vi "Test Variant to Objects.vi"() -> ()   [LabVIEW 2021]
uses:
  Source/Support/Nodes/Leaves/Synch/With Values/WaitOn/bt_WaitOn_Synch_WithValues.lvclass
  <vilib>/ErrorRing/Error Ring.xnode
  <vilib>/Utility/error.llb/Error Cluster From Error Code.vi
  <vilib>/measure/NI_MABase.lvlib
  <vilib>/TSA/Abstract Data Classes/Abs_Types/Waveform/Abs_Waveform.lvclass
  <vilib>/TSA/Abstract Data Classes/Abs_Types/Boolean/Abs_Boolean.lvclass
  <vilib>/TSA/Abstract Data Classes/Abs_Types/I32 Integer/Abs_I32 Integer.lvclass
  <vilib>/TSA/Abstract Data Classes/Abs_Types/String/Abs_String.lvclass
  <vilib>/TSA/Omni-Bus/Local Bus/Local Bus.lvclass
  <vilib>/Utility/Data Type/Type Definitions/Data Type.ctl
  <vilib>/Utility/Data Type/NI_Data Type.lvlib
  <vilib>/TSA/Omni-Bus/Local Bus/Support/Tag List Type.ctl
  <vilib>/TSA/Omni-Bus/Omni-Bus/Omni_Bus.lvclass
  <vilib>/TSA/Abstract Data Classes/Abs_Types/Double Float/Abs_Double Float.lvclass
  <vilib>/TSA/Omni-Bus/Omni-Bus/Support/Get/Get DBL.vi
  <vilib>/TSA/Abstract Data Classes/Abs_Types/Time/Abs_Time.lvclass
  <vilib>/TSA/Abstract Data Classes/Abs_Types/Boolean/Simple Read.vi
  <vilib>/TSA/Abstract Data Classes/Abs_Types/I32 Integer/Simple Read.vi
  <vilib>/TSA/Abstract Data Classes/Abs_Types/String/Simple Read.vi
  <vilib>/TSA/Abstract Data Classes/Abs_Types/Waveform/Simple Read.vi
  <vilib>/TSA/Abstract Data Classes/Abs_Types/Time/Simple Read.vi
  <vilib>/TSA/Omni-Bus/Omni-Bus/Support/Write/Write DBL.vi
  <vilib>/TSA/Abstract Data Classes/Abs_Types/Double Float/Simple Read.vi
  C:/Program Files (x86)/National Instruments/LabVIEW 2021/vi.lib/TSA/Omni-Bus/Omni-Bus/Bus Access/Bus_Access.lvclass
  C:/Program Files (x86)/National Instruments/LabVIEW 2021/vi.lib/TSA/Abstract Data Classes/Abs_Types/Type/Abs_Type.lvclass
  C:/Program Files (x86)/National Instruments/LabVIEW 2021/vi.lib/TSA/Omni-Bus/Local Bus/Local Bus.lvclass
  <vilib>/TSA/Abstract Data Classes/Abs_Types/Value/Abs_Value.lvclass
  <vilib>/TSA/Abstract Data Classes/Abs_Types/Time/Support/Type.ctl
panel:
  out "Value 3":T1
  out "current time":timestamp
  in  "Numeric":dbl
  in  "stop":bool
  out "Value 2":dbl
  out "String":string
  out "Value":i32
  out "Boolean":bool
  out "Waveform Graph":waveform(dbl)(graph)
  out "Names OUT":string[](array[string])
  out "Value Objects OUT":refnum<class "Abs_Value.lvclass">[](array[class])
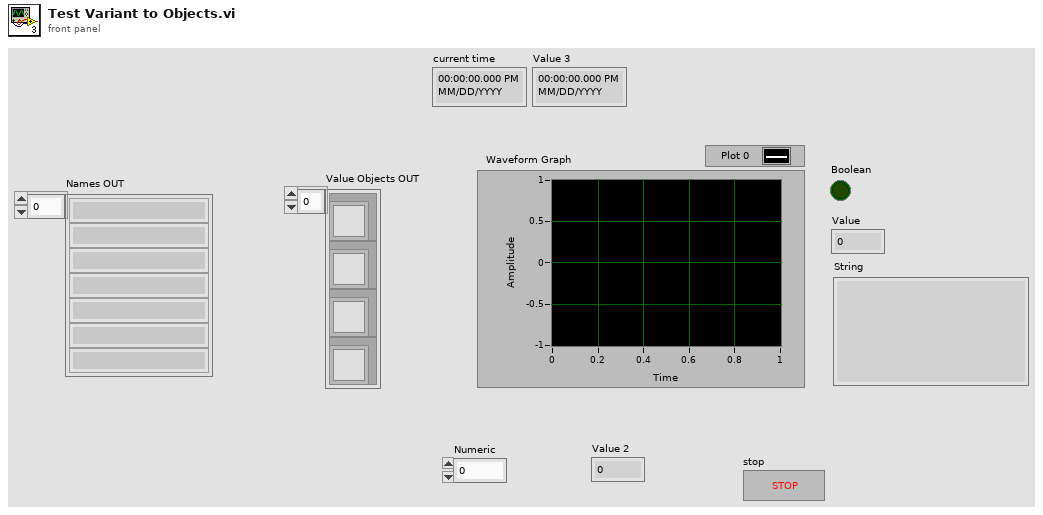
[diagram p1: front panel]
types:
  T1 = typedef "Abs_Time.lvclass/Type.ctl" = timestamp
  T2 = typedef "Local Bus.lvclass/Tag List Type.ctl" = cluster{"Tag":string, "Type":T3}
  T3 = typedef "NI_Data Type.lvlib/Data Type.ctl" = enum8{"Invalid Type", "Void", "I8", "I16", "I32", "I64", "U8", "U16", "U32", "U64", "Single Float", "Double Float", "Extended Float", "Single Complex", "Double Complex", "Extended Complex", "Enum U8", "Enum U16", "Enum U32", "Enum U64", "Single Float With Unit", "Double Float With Unit", "Extended Float With Unit", "Single Complex with Unit", "Double Complex with Unit", "Extended Complex with Unit", "Boolean", "String", "Path", "Picture", "Tag", "Array", "Cluster", "Variant", "LV Variant", "Waveform", "Timestamp", "Digital Waveform", "Digital Data", "ExpressData", "Refnum", "External Data", "VI", "Poly VI", "LabVIEW Class Instance", "Fixed Point", "Set Collection", "Map Collection"}
  T4 = cluster{"signal out":waveform(dbl), "error out":errorcluster, "Value Out":refnum<class "Abs_Double Float.lvclass">, "seconds since 1Jan1904":timestamp}
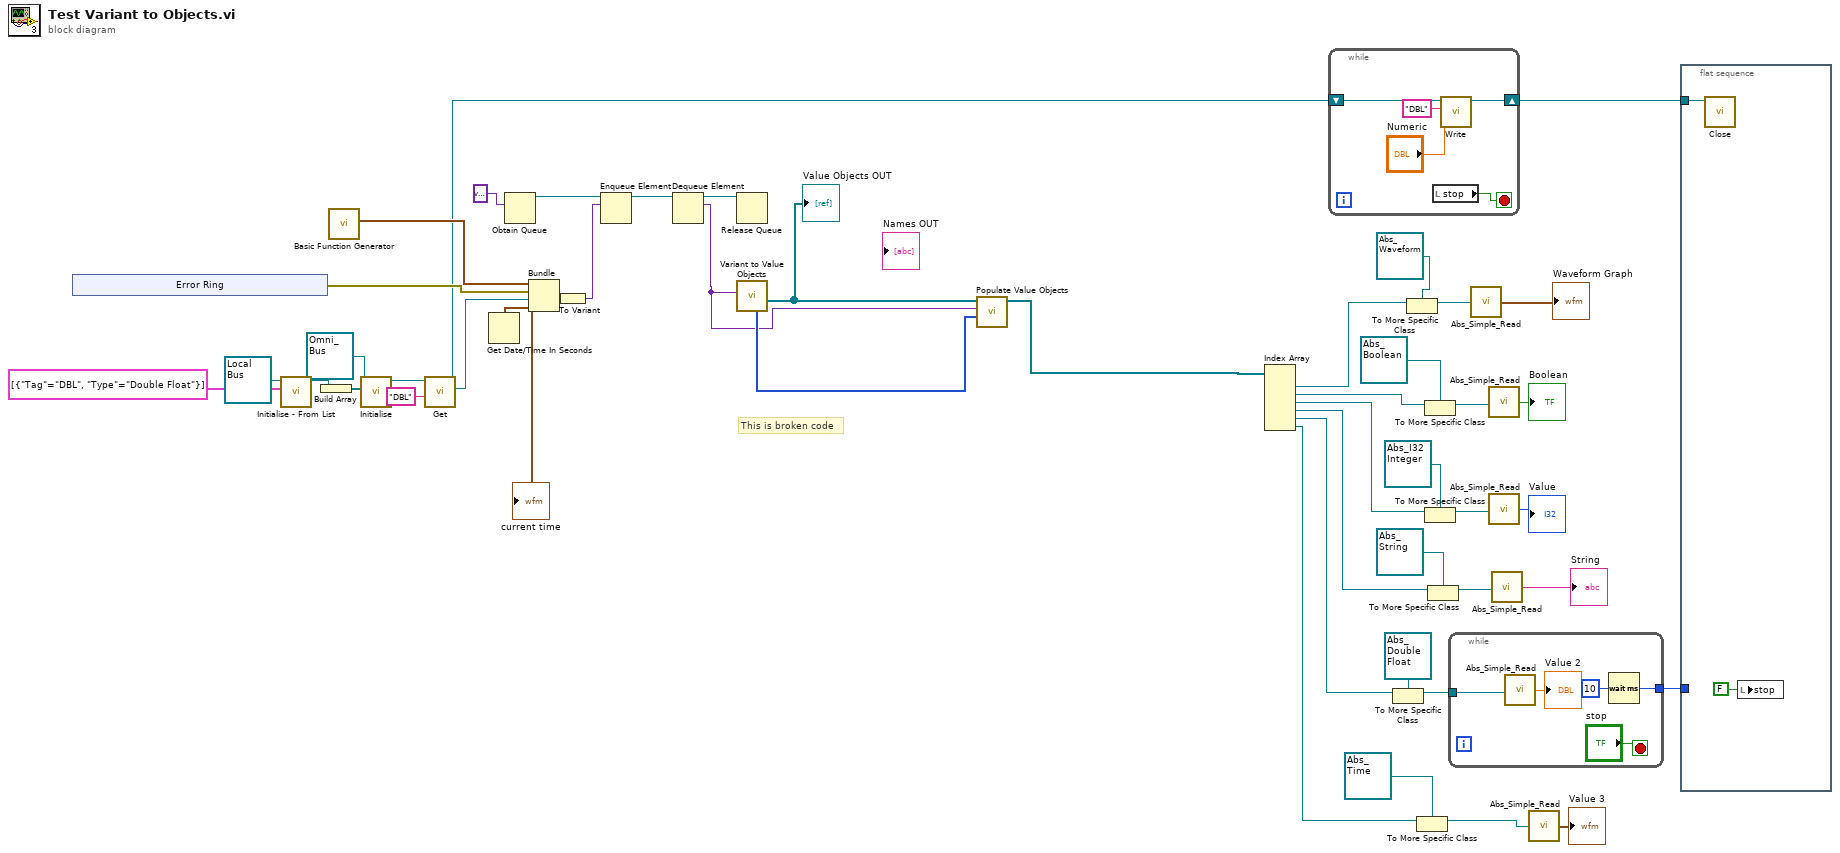
[diagram p0: block diagram]
diagram:
  # "This is broken code"
  n1 = xnode "Error Ring"() -> ("error out"=w46:errorcluster)
  n2 = call <vilib>:"Initialise - From List.vi"("Tag List"=T2[] [{"Tag"="DBL", "Type"=enum."Double Float"}], "Local Bus in"=refnum<class "Local Bus.lvclass"> refnum) -> ("Local Bus out"=w26:refnum<class "Local Bus.lvclass">)  [unwired: 8 in, 1 out]
  n3 = Build Array(w26) -> (w25:refnum<class "Local Bus.lvclass">[])
  n4 = call <vilib>:"Basic Function Generator.vi"() -> ("signal out"=w45:waveform(dbl))  [unwired: 9 in, 2 out]
  n5 = call-dynamic "Initialise.vi"("Bus Access"=w25, "Var Bus in"=refnum<class "Omni_Bus.lvclass"> refnum) -> ("Var Bus out"=w23:refnum<class "Omni_Bus.lvclass">)  [unwired: 8 in, 1 out]
  n6 = call-poly <vilib>:"Get.vi"("Tag"="DBL", "Var Bus in"=w23) -> ("Value Out"=w21:refnum<class "Abs_Double Float.lvclass">, "Var Bus out"=w17:refnum<class "Omni_Bus.lvclass">)  [unwired: 6 in, 2 out]
  n7 = Get Date/Time In Seconds() -> (seconds since 1Jan1904=w14:timestamp)
  "current time" <- w14
  n8 = Obtain Queue(element data type=variant) -> (queue out=w8:refnum<queue>)  [unwired: 4 in, 2 out]
  n9 = Bundle("signal out"=w45, "error out"=w46, "Value Out"=w21, "seconds since 1Jan1904"=w14) -> (w47:T4)  [unwired: 1 in]
  n10 = To Variant(anything=w47) -> (Variant=w7:variant)
  n11 = Enqueue Element(queue=w8, element=w7) -> (queue out=w5:refnum<queue>)  [unwired: 2 in, 2 out]
  n12 = Dequeue Element(queue=w5) -> (queue out=w6:refnum<queue>, element=w1:variant)  [unwired: 2 in, 2 out]
  n13 = Release Queue(queue=w6) -> ()  [unwired: 2 in, 3 out]
  n14 = call "Variant to Value Objects.vi"("Variant"=w1) -> ("Value Objects OUT"=w4:refnum<class "Abs_Value.lvclass">[], "types out"=w3:T3[])  [unwired: 7 in, 2 out]
  "Value Objects OUT" <- w4
  n15 = call "Populate Value Objects.vi"("LabVIEW types"=w3, "Variant"=w1, "Value Objects Type"=w4) -> ("Value Objects Out"=w2:refnum<class "Abs_Value.lvclass">[])  [unwired: 7 in, 1 out]
  n16 = Index Array(array=w2) -> (element #1=w44:refnum<class "Abs_Value.lvclass">, element #2=w40:refnum<class "Abs_Value.lvclass">, element #3=w35:refnum<class "Abs_Value.lvclass">, element #4=w33:refnum<class "Abs_Value.lvclass">, element #5=w18:refnum<class "Abs_Value.lvclass">, element #6=w13:refnum<class "Abs_Value.lvclass">)  [unwired: 6 in]
  n17 = while {
    shift-right: [w51] -> w15
    shift-left: w17 -> [w52]
    stop <- w48 stop-if-true
    n18 = local read "stop"() -> (w48:bool)
    n19 = call-poly <vilib>:"Write.vi"("Numeric"="Numeric", "Tag"="DBL", "Omni_Bus in"=w52) -> ("Omni_Bus out"=w51:refnum<class "Omni_Bus.lvclass">)  [unwired: 7 in, 1 out]
  }
  n20 = To More Specific Class(target class=refnum<class "Abs_Double Float.lvclass"> refnum ("Class"), reference=w18) -> (specific class reference=w19:refnum<class "Abs_Double Float.lvclass">)  [unwired: 1 in, 1 out]
  n21 = To More Specific Class(target class=refnum<class "Abs_Waveform.lvclass"> refnum ("Abs_Waveform in"), reference=w44) -> (specific class reference=w42:refnum<class "Abs_Waveform.lvclass">)  [unwired: 1 in, 1 out]
  n22 = To More Specific Class(target class=refnum<class "Abs_Time.lvclass"> refnum ("Class"), reference=w13) -> (specific class reference=w11:refnum<class "Abs_Time.lvclass">)  [unwired: 1 in, 1 out]
  n23 = To More Specific Class(target class=refnum<class "Abs_Boolean.lvclass"> refnum ("Boolean in"), reference=w40) -> (specific class reference=w39:refnum<class "Abs_Boolean.lvclass">)  [unwired: 1 in, 1 out]
  n24 = To More Specific Class(target class=refnum<class "Abs_I32 Integer.lvclass"> refnum ("Class"), reference=w35) -> (specific class reference=w36:refnum<class "Abs_I32 Integer.lvclass">)  [unwired: 1 in, 1 out]
  n25 = To More Specific Class(target class=refnum<class "Abs_String.lvclass"> refnum ("Abs_String in"), reference=w33) -> (specific class reference=w34:refnum<class "Abs_String.lvclass">)  [unwired: 1 in, 1 out]
  n26 = while {
    tunnel: w19 -> [w54]
    tunnel: [w53] -> w16
    stop <- "stop" stop-if-true
    n27 = call-poly <vilib>:"Abs_Simple_Read.vi"("Class"=w54) -> ("Value"=→"Value 2":dbl)  [unwired: 4 in]
    n28 = Wait (ms)(milliseconds to wait=u32 10) -> (millisecond timer value=w53:u32)
  }
  n29 = call-poly <vilib>:"Abs_Simple_Read.vi"("Abs_Waveform in"=w42) -> ("Waveform"=→"Waveform Graph":waveform(dbl))  [unwired: 4 in]
  n30 = call-poly <vilib>:"Abs_Simple_Read.vi"("Boolean in"=w39) -> ("Boolean"=→"Boolean":bool)  [unwired: 4 in]
  n31 = call-poly <vilib>:"Abs_Simple_Read.vi"("Class"=w36) -> ("Value"=→"Value":i32)  [unwired: 4 in]
  n32 = call-poly <vilib>:"Abs_Simple_Read.vi"("Abs_String in"=w34) -> ("String"=→"String":string)  [unwired: 4 in]
  n33 = call-poly <vilib>:"Abs_Simple_Read.vi"("Class"=w11) -> ("Value"=→"Value 3":T1)  [unwired: 4 in]
  n34 = flat-sequence {
    tunnel: w16 -> [_]
    tunnel: w15 -> [w59]
    frame #0 {
      n35 = call-dynamic "Close.vi"("Data in"=w59) -> ()  [unwired: 9 in, 2 out]
      n36 = local write "stop"(FALSE ("stop")) -> ()
    }
  }
